vi "03-without_args_and_returned_val.vi"() -> ()   [LabVIEW 2018, in "LV2Julia_examples.lvlib"]
uses:
  LV2Julia_examples.lvlib
  LV2Julia_core/VIs/Server or client state.ctl
  LV2Julia_core/VIs/detailed error info.ctl
  LV2Julia_core/VIs/StackFrame.ctl
  LV2Julia_core/VIs/Commands.ctl
  3a82b6dd-e193-42c5-8b03-f24c274193dd.vi
  3a82b6dd-e193-42c5-8b03-f24c274193dd.vi/5bdd2d35-9a1a-447e-993c-fa423b711998.vi
  3a82b6dd-e193-42c5-8b03-f24c274193dd.vi/5bdd2d35-9a1a-447e-993c-fa423b711998.vi/e7ce0a4e-8fc1-4c02-ab50-bb243ed617e9.vi
  3a82b6dd-e193-42c5-8b03-f24c274193dd.vi/5bdd2d35-9a1a-447e-993c-fa423b711998.vi/469a2b6c-b6b1-4aed-b403-0ad2eeee620a.vi
  3a82b6dd-e193-42c5-8b03-f24c274193dd.vi/5bdd2d35-9a1a-447e-993c-fa423b711998.vi/68d586c8-cd2d-43f8-8e7c-70015861bd16.vi
  LV2Julia_core/VIs/jl-scripts path.vi
  LV2Julia_core/VIs/check ID validity.vi
  LV2Julia_core/VIs/bindata_descr to JSON.vi
  LV2Julia_core/VIs/check cluster field names.vi
  LV2Julia_core/VIs/concat JSON.vi
  LV2Julia_core/VIs/build request.vi
  LV2Julia_core/VIs/Parse server response.vi
  LV2Julia_core/VIs/log jl exceptions.vi
  LV2Julia_core/LV2Julia_core.lvlib
panel:
  in  "next":bool
  out "detailed error info":T1
  out "current error":errorcluster
  out "final error":errorcluster
  out "short err code":u8
  in  "stop":bool
  out "ZMQ timeout":bool
  out "Julia script file path":path
  out "temporary script path":path
  out "Jl Server state":T3
  # "No arguments are sent and no values recieved here. The Julia script should each time print \"Hello World!\" in the terminal window."
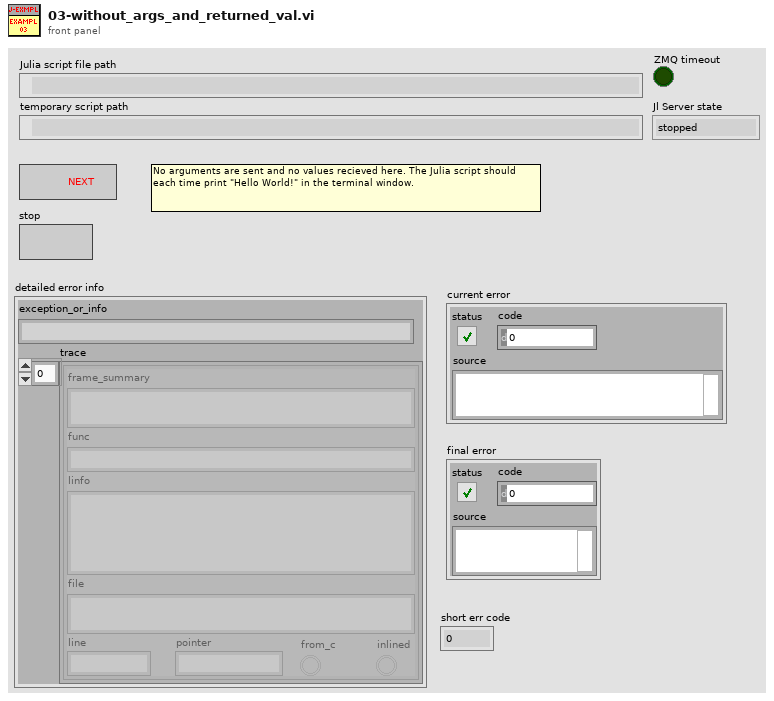
[diagram p1: front panel]
types:
  T1 = typedef "LV2Julia_core.lvlib/detailed error info.ctl" = cluster{"exception_or_info":string, "trace":T2[]}
  T2 = typedef "LV2Julia_core.lvlib/StackFrame.ctl" = cluster{"frame_summary":string, "func":string, "linfo":string, "file":string, "line":i32, "pointer":u64, "from_c":bool, "inlined":bool}
  T3 = typedef "LV2Julia_core.lvlib/Server or client state.ctl" = enum16{"stopped", "running", "unknown"}
  T4 = typedef "LV2Julia_core.lvlib/Commands.ctl" = enum16{"Start Jl-server & Init LV-client", "Send request & Get response ", "Stop Jl-server & Cleanup LV-client", "Cleanup LV-client", "Start Jl-server", "Stop Jl-server", "Init LV-Client", "Cleanup LV-Client", "(not allowed)", "Set LV Client state", "Set Jl Server state", "set ZMQ timeout", "read ZMQ timeout", "read-out state"}
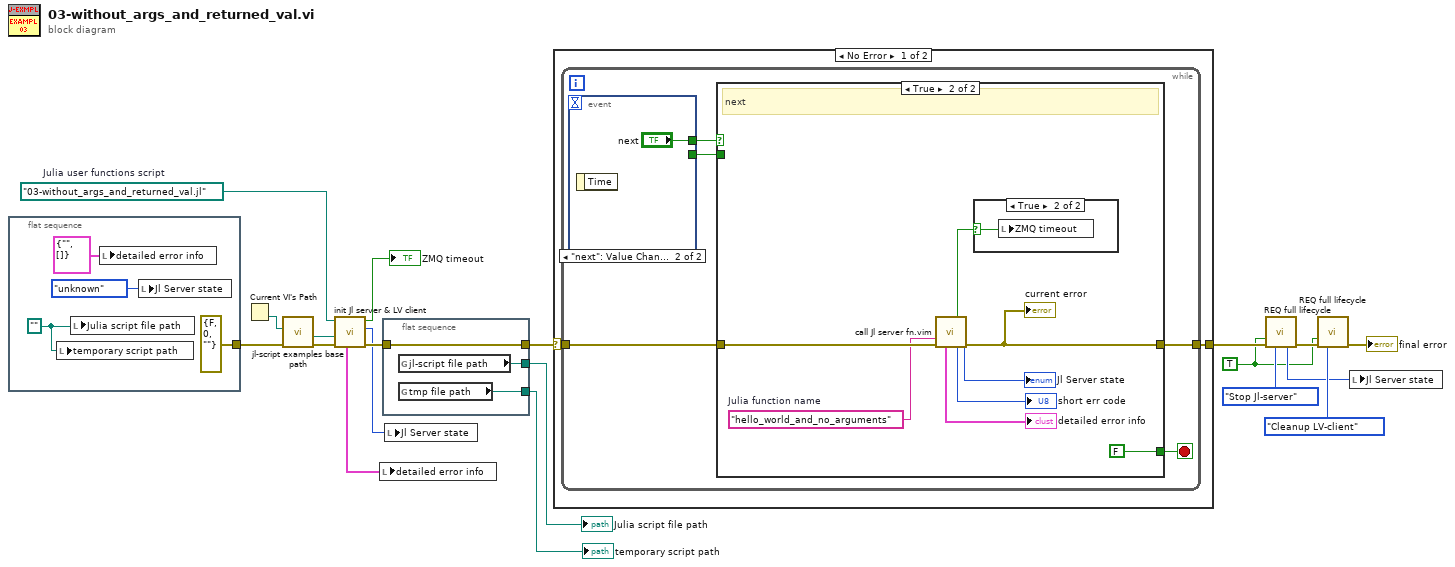
[diagram p0: block diagram]
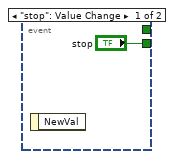
[diagram p2: hidden frame]
diagram:
  w9 = path "03-without_args_and_returned_val.jl"  # Julia user functions script
  w10 = TRUE ("Force command")
  n1 = flat-sequence {
    tunnel: [errorcluster {"status"=FALSE, "code"=0, "source"=""} ("error in (no error)")] -> w2
    frame #0 {
      w20 = path ""
      n2 = local write "temporary script path"(w20) -> ()
      n3 = local write "Julia script file path"(w20) -> ()
      n4 = local write "detailed error info"(T1 {"exception_or_info"="", "trace"=[]} ("detailed error info")) -> ()
      n5 = local write "Jl Server state"(Server_or_client_state."unknown" ("Jl Server state out")) -> ()
    }
  }
  n6 = Current VI's Path() -> (path=w5:path)
  n7 = call "jl-script examples base path.vi"("error in (no error)"=w2, "calling example VI path"=w5) -> ("error out"=w4:errorcluster, "jl-script-examples base path"=w3:path)  [unwired: 8 in]
  n8 = call "init Jl server & LV client.vi"("error in (no error)"=w4, "Base path (not a path)"=w3, "Julia user functions script"=w9) -> ("error out"=w8:errorcluster, "Jl Server state out"=w6:T3, "timeout?"=→"ZMQ timeout":bool, "detailed error info"=w1:T1)  [unwired: 3 in, 2 out]
  n9 = local write "detailed error info"(w1) -> ()
  n10 = flat-sequence {
    tunnel: [w26] -> w14
    tunnel: w8 -> [w26]
    tunnel: [w25] -> w12
    tunnel: [w24] -> w13
    frame #0 {
      n11 = global read "jl-scripts path.vi" "jl-script file path"() -> (w25:path)
      n12 = global read "jl-scripts path.vi" "tmp file path"() -> (w24:path)
    }
  }
  n13 = local write "Jl Server state"(w6) -> ()
  n14 = case shown="No Error" w14 {
    selector: w14 -> [w27 w47]
    tunnel: [w28 w47] -> w19
    frame No Error {
      n15 = while {
        tunnel: w27 -> [w32]
        tunnel: [w33] -> w28
        stop <- w30 stop-if-true
        n16 = event shown="[1] \"next\": Value Change" {
          selector: _ -> [_ _]
          dyn-events: _ -> [_ _]
          timeout: _ -> [_ _]
          tunnel: [_ "next"] -> w31
          tunnel: ["stop" _] -> w29
          event "stop": Value Change {
            n17 = event-data() -> ()  [unwired: 1 in, 1 out]
          }
          event "next": Value Change {
            n18 = event-data() -> ()  [unwired: 1 in, 1 out]
          }
        }
        n19 = case shown="True" w31 {
          tunnel: [w37 w43] -> w33
          tunnel: w32 -> [w37 w44]
          tunnel: [w36 FALSE ("stop this VI only")] -> w30
          tunnel: w29 -> [w36 _]
          frame False {
            # "stop"
          }
          frame True {
            w41 = "hello_world_and_no_arguments"  # Julia function name
            # "next"
            n20 = call "call Jl server fn.vim"("fun2call"=w41, "error in (no error)"=w44) -> ("timeout?"=w42:bool, "Jl Server state out"=→"Jl Server state":T3, "detailed error info"=→"detailed error info":T1, "return code"=→"short err code":u8, "error out"=w43:errorcluster)  [unwired: 7 in, 2 out]
            "current error" <- w43
            n21 = case shown="True" w42 {
              selector: w42 -> [_ w46]
              frame False {
              }
              frame True {
                n22 = local write "ZMQ timeout"(w46) -> ()
              }
            }
          }
        }
      }
    }
    frame Error {
    }
  }
  n23 = call "REQ full lifecycle.vi"("Force command"=w10, "error in"=w19, "command"=Commands."Stop Jl-server") -> ("Jl Server state out"=w11:T3, "error out"=w17:errorcluster)  [unwired: 6 in, 5 out]
  n24 = call "REQ full lifecycle.vi"("Force command"=w10, "error in"=w17, "command"=Commands."Cleanup LV-client") -> ("error out"=→"final error":errorcluster)  [unwired: 6 in, 6 out]
  n25 = local write "Jl Server state"(w11) -> ()
  "temporary script path" <- w13
  "Julia script file path" <- w12
